vi "File Age Rollover.vi"() -> ()   [LabVIEW 2018]
uses:
  9011d6f2-2c15-4807-9024-144d7f9aaf38.vi
  d03bfca0-c32b-4c69-80d4-a3e8b21c997e.vi
  9011d6f2-2c15-4807-9024-144d7f9aaf38.vi/0a1ee2ab-da6d-4243-8cf3-8125e611a602.vi
  src/api/Log.vi
  src/api/configuration/handlers/file_handler/RolloverTrigger.Age/RolloverTrigger.Age.lvclass
  C:/Users/Colin/Documents/software_projects/labview/glog/src/api/configuration/handlers/file_handler/RolloverTrigger/RolloverTrigger.lvclass
  src/api/configuration/handlers/file_handler/File Handler.lvclass
  C:/Users/Colin/Documents/software_projects/labview/glog/src/api/extension/formatting_handler_interface/Formatting Handler.lvclass
  src/api/configuration/handlers/file_handler/New (Single Trigger).vi
  src/registry/Log.vi
  src/api/GLog.lvlib
panel:
  in  "rollover age [s]":dbl=1.0 format="%#_13g"
  out "error out":errorcluster
  in  "Stop":bool
  out "Current Log File":path
  out "Source":string
  out "log files":path[](array[path])
  out "sources":string[](array[string])
  in  "runtime [s]":dbl=3.0 format="%#_13g"
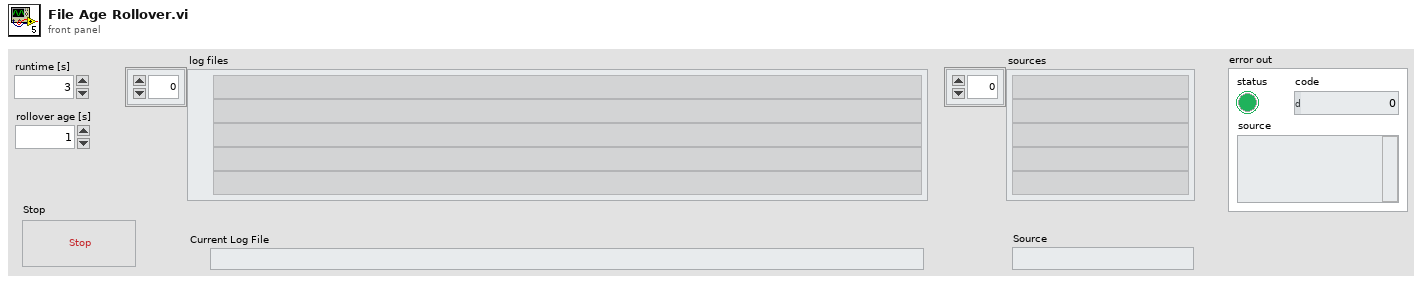
[diagram p1: front panel]
types:
  T1 = typedef "GLog.lvlib/File Handler.lvclass/Events.ctl" = cluster{"File Rollover":refnum<user-event>}
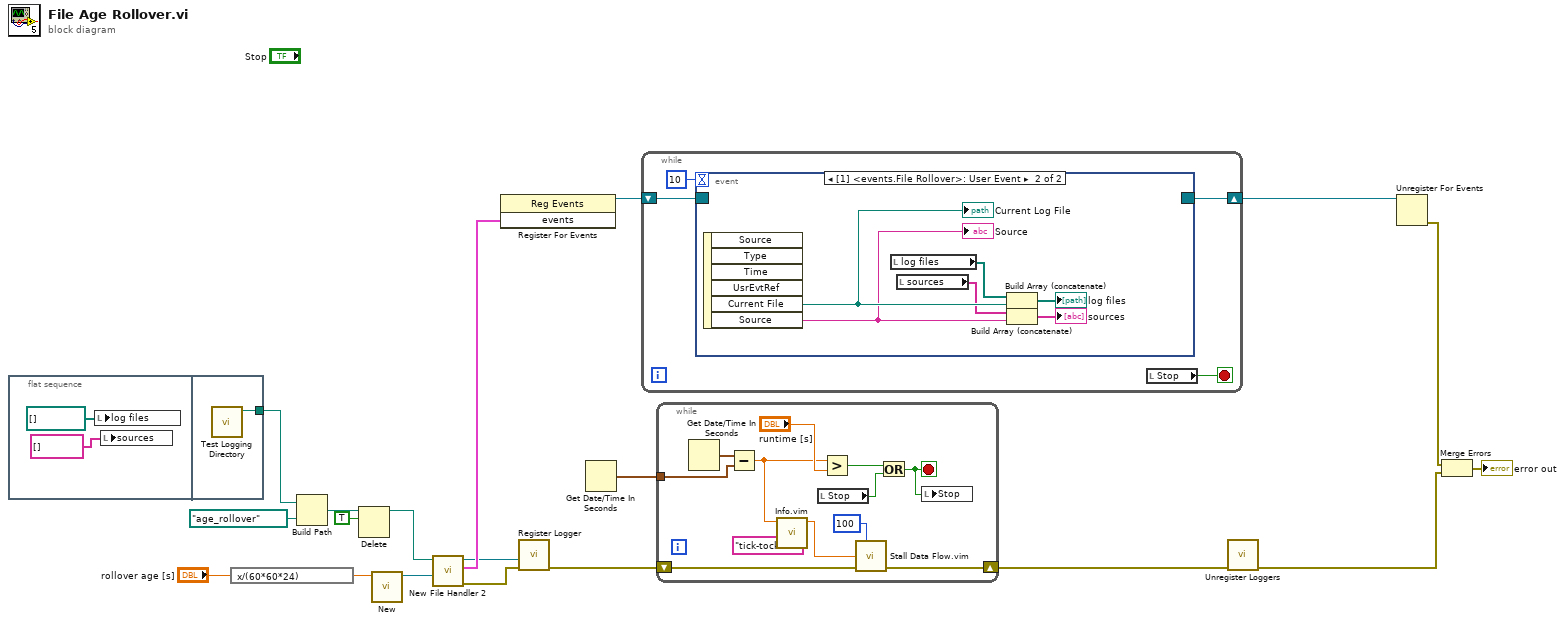
[diagram p0: block diagram]
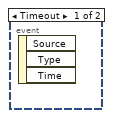
[diagram p2: hidden frame]
diagram:
  n1 = flat-sequence {
    tunnel: [w22] -> w1
    frame #0 {
      n2 = local write "log files"(path[] [] ("log files")) -> ()
      n3 = local write "sources"(string[] [] ("sources")) -> ()
    }
    frame #1 {
      n4 = call "Test Logging Directory.vi"() -> ("test logging directory"=w22:path)  [unwired: 11 in]
    }
  }
  n5 = expression code="x/(60*60*24)"("rollover age [s]") -> (w14:dbl)
  n6 = Build Path(base path=w1, name or relative path=path "age_rollover") -> (appended path=w18:path)
  n7 = Delete(path (use dialog)=w18, entire hierarchy (F)=TRUE) -> (deleted path=w13:path)  [unwired: 3 in, 2 out]
  n8 = call "New.vi"("age limit (1)[days]"=w14) -> ("RolloverTrigger.Age"=w16:refnum<class "RolloverTrigger.Age.lvclass">)  [unwired: 10 in]
  n9 = call-poly "New File Handler 2.vi"("rollover trigger (50 MB)"=w16, "log directory (<app dir>/logs)"=w13) -> ("error out"=w3:errorcluster, "events"=w9:T1, "file handler"=w2:refnum<class "File Handler.lvclass">)  [unwired: 7 in]
  n10 = register-events(w9) -> (reference out=w11:refnum<event-registration>)  [unwired: 2 in, 1 out]
  n11 = call "Register Logger.vi"("error in (no error)"=w3, "log handler (file handler)"=w2) -> ("error out"=w4:errorcluster)  [unwired: 9 in]
  n12 = Get Date/Time In Seconds() -> (seconds since 1Jan1904=w12:timestamp)
  n13 = while {
    shift-right: [w25] -> w10
    shift-left: w11 -> [w26]
    stop <- w24 stop-if-true
    n14 = event shown="[1] <events.File Rollover>: User Event" {
      selector: w26 -> [_ _]
      dyn-events: [_ _] -> w25
      timeout: 10 -> [_ _]
      event Timeout {
        n15 = event-data() -> ()  [unwired: 1 in, 3 out]
      }
      event User Event {
        n16 = event-data() -> ("Current File"=w32:path, "Source"=w31:string)  [unwired: 1 in, 4 out]
        "Current Log File" <- w32
        "Source" <- w31
        n17 = local read "log files"() -> (w28:path[])
        n18 = local read "sources"() -> (w27:string[])
        n19 = Build Array (concatenate)(w28, w32) -> (→"log files":path[])
        n20 = Build Array (concatenate)(w27, w31) -> (→"sources":string[])
      }
    }
    n21 = local read "Stop"() -> (w24:bool)
  }
  n22 = while {
    tunnel: w12 -> [w43]
    shift-right: [w36] -> w7
    shift-left: w4 -> [w36]
    stop <- w34 stop-if-true
    n23 = Get Date/Time In Seconds() -> (seconds since 1Jan1904=w42:timestamp)
    n24 = Subtract(x=w42, y=w43) -> (x-y=w39:dbl)
    n25 = call "Info.vim"("data in (null)"=w39, "message"="tick-tock") -> ("data out"=w38:dbl)  [unwired: 9 in]
    n26 = local read "Stop"() -> (w33:bool)
    n27 = Greater?(x=w39, y="runtime [s]") -> (0:w35:bool)
    n28 = call "Stall Data Flow.vim"("value in"=w38, "milliseconds to wait"=u32 100) -> ()  [unwired: 2 out]
    n29 = Or(x=w35, y=w33) -> (x .or. y?=w34:bool)
    n30 = local write "Stop"(w34) -> ()
  }
  n31 = call "Unregister Loggers.vi"("error in (no error)"=w7) -> ("error out"=w5:errorcluster)  [unwired: 9 in, 1 out]
  n32 = Unregister For Events(event registration refnum=w10) -> (error out=w8:errorcluster)  [unwired: 1 in]
  n33 = Merge Errors(w8, w5) -> (→"error out":errorcluster)
